vi "Output CAN Message Command to Main.vi"(8 "error in (no error)":errorcluster, 10 "Output Message":u8[](array[numeric]), 11 "CIFPlugin in":refnum<class "CAN_Writer_NIXNET_Plugin.lvclass">) -> (0 "error out":errorcluster, 3 "CIFPlugin out":refnum<class "CAN_Writer_NIXNET_Plugin.lvclass">)   [LabVIEW 2021, in "CAN_Writer_NIXNET_Plugin.lvclass"]
uses:
  CAN_Writer_NIXNET_Plugin.lvclass
  CAN_Writer_NIXNET_Plugin.lvclass/CAN_Writer_NIXNET_Plugin.ctl
  Common/Typedef/OOB Comm/To Main DVR Data.ctl
  Common/Typedef/OOB Comm/To Main Command Payload.ctl
  Common/Typedef/OOB Comm/To Main Command.ctl
  Common/Typedef/OOB Comm/To Main Command Data.ctl
  cb651c69-5256-45bc-b9b0-1818fa9c55ac.vi
  <vilib>/CIF Foundation/CIF CIPC/SubVIs/Check Error.vi
  <vilib>/CIF Foundation/CIF CIPC/SubVIs/Notify Of New Write.vi
  <vilib>/CIF Foundation/CIF CIPC/SubVIs/Get dll Path.vi
  <vilib>/CIF Foundation/CIF CIPC/SubVIs/Get Element Write Position.vi
  <vilib>/CIF Foundation/CIF CIPC/SubVIs/Get Element Info Variant.vi
  <vilib>/CIF Foundation/CIF CIPC/SubVIs/Check Error Core.vi
  8779bfbf-2797-4940-8d62-f4162e828731.vi
  Common/CAN_Writer_NIXNET_Common.lvlib
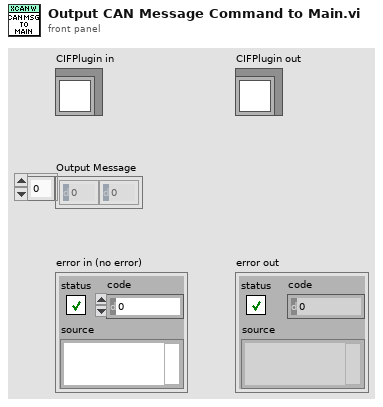
[diagram p1: front panel]
types:
  T1 = typedef "CAN_Writer_NIXNET_Common.lvlib/To Main DVR Data.ctl" = cluster{"Data 1 DVR  -> Main":i32, "Output Message":u8[]}
  T2 = typedef "CAN_Writer_NIXNET_Common.lvlib/To Main Command Payload.ctl" = cluster{"Command":T3, "-> Main":T4}
  T3 = typedef "CAN_Writer_NIXNET_Common.lvlib/To Main Command.ctl" = enum16{"Read Data", "Read DVR Data", "Output Message"}
  T4 = typedef "CAN_Writer_NIXNET_Common.lvlib/To Main Command Data.ctl" = cluster{"Cmd Data 1 -> Main":i32}
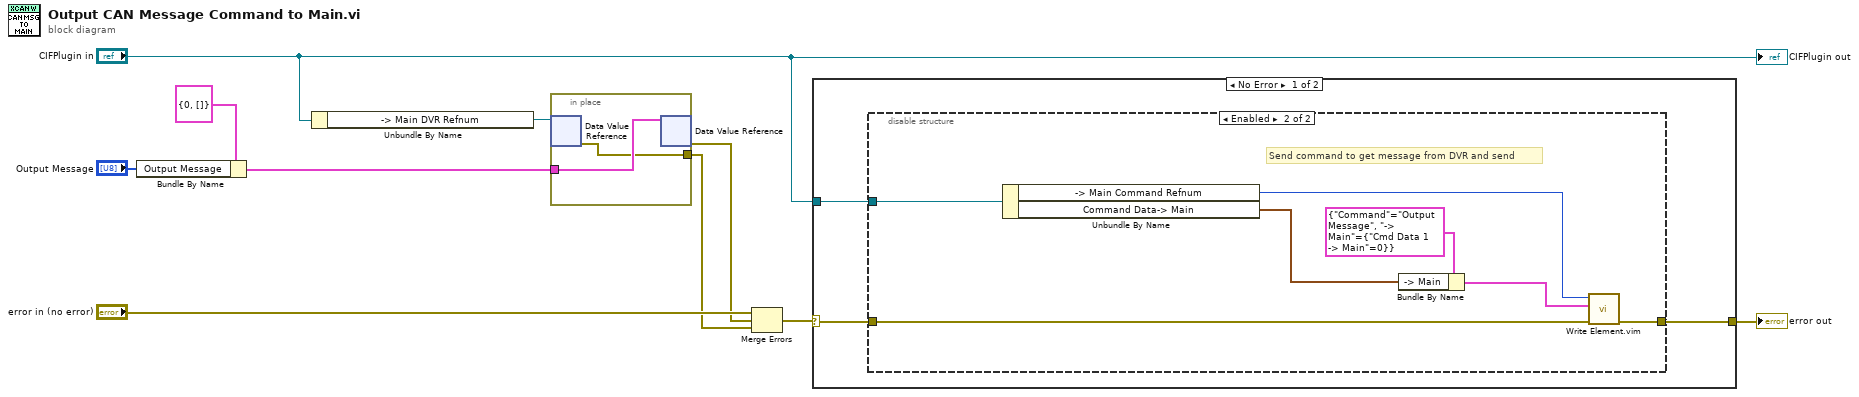
[diagram p0: block diagram]
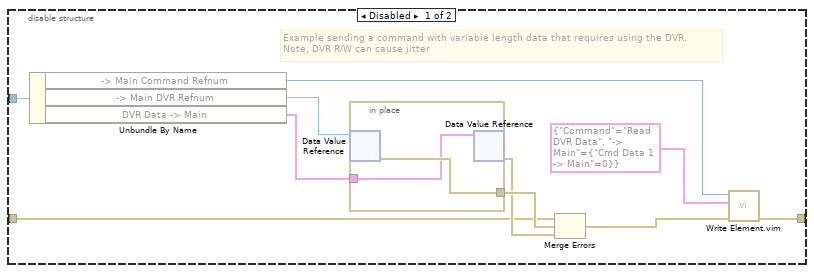
[diagram p2: hidden frame]
diagram:
  n1 = Bundle By Name(cluster=T1 {"Data 1 DVR  -> Main"=0, "Output Message"=[]} ("-> Main Comm.DVR Data -> Main"), "Output Message"="Output Message") -> (w7:T1)
  n2 = Unbundle By Name("CIFPlugin in") -> ("-> Main DVR Refnum"=w5:refnum<data-value>)
  n3 = in-place {
    in-place-border: w7 -> [w12]
    in-place-border: [w11] -> w2
    n4 = in-place-dvr #1(w5) -> (w11:errorcluster)  [unwired: 1 out]
    n5 = in-place-dvr #1(w12) -> (w1:errorcluster)  [unwired: 1 out]
  }
  n6 = Merge Errors("error in (no error)", w1, w2) -> (w3:errorcluster)
  n7 = case shown="No Error" w3 {
    selector: w3 -> [w14 w35]
    tunnel: [w13 w35] -> w10
    tunnel: "CIFPlugin in" -> [w15 _]
    frame No Error {
      n8 = disable-structure shown="Enabled" {
        disable-tunnel: w15 -> [w20 w33]
        disable-tunnel: w14 -> [w19 w31]
        disable-tunnel: [w18 w32] -> w13
        frame Disabled {
          # "Example sending a command with variable length data that requires using the DVR.\nNote, DVR R/W can cause jitter"
          n9 = Unbundle By Name(w20) -> ("-> Main Command Refnum"=w22:u64, "-> Main DVR Refnum"=w25:refnum<data-value>, "DVR Data -> Main"=w16:T1)
          n10 = in-place {
            in-place-border: [w27] -> w23
            in-place-border: w16 -> [w26]
            n11 = in-place-dvr #2(w25) -> (w27:errorcluster)  [unwired: 1 out]
            n12 = in-place-dvr #2(w26) -> (w21:errorcluster)  [unwired: 1 out]
          }
          n13 = Merge Errors(w19, w23, w21) -> (w24:errorcluster)
          n14 = call "Write Element.vim"("error in (no error)"=w24, "Data in"=T2 {"Command"=enum."Read DVR Data", "-> Main"={"Cmd Data 1 -> Main"=0}} ("Payload"), "CIPC Reference in"=w22) -> ("error out"=w18:errorcluster)  [unwired: 5 in, 3 out]
        }
        frame Enabled {
          # "Send command to get message from DVR and send"
          n15 = Unbundle By Name(w33) -> ("-> Main Command Refnum"=w34:u64, "Command Data-> Main"=w28:T4)
          n16 = Bundle By Name(cluster=T2 {"Command"=enum."Output Message", "-> Main"={"Cmd Data 1 -> Main"=0}} ("Payload"), "-> Main"=w28) -> (w29:T2)
          n17 = call "Write Element.vim"("error in (no error)"=w31, "Data in"=w29, "CIPC Reference in"=w34) -> ("error out"=w32:errorcluster)  [unwired: 5 in, 3 out]
        }
      }
    }
    frame Error {
    }
  }
  "error out" <- w10
  "CIFPlugin out" <- "CIFPlugin in"
